vi "Make String Mermaid Safe.vi"(11 "Source CSM":string) -> (3 "result string":string)   [LabVIEW 2020, in "CSM Mermaid Support.lvlib"]
uses:
  CSM Mermaid Support.lvlib
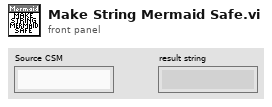
[diagram p1: front panel]
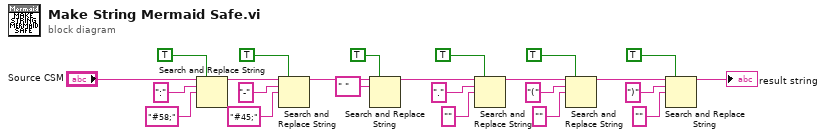
[diagram p0: block diagram]
diagram:
  n1 = Search and Replace String(replace all?=TRUE ("replace all? (F)"), input string="Source CSM", search string=":", replace string="#58;" ("search string")) -> (result string=w17:string)  [unwired: 4 in, 3 out]
  n2 = Search and Replace String(replace all?=TRUE ("replace all? (F)"), input string=w17, search string="-", replace string="#45;" ("search string")) -> (result string=w2:string)  [unwired: 4 in, 3 out]
  n3 = Search and Replace String(replace all?=TRUE ("replace all? (F)"), input string=w2, search string=" ") -> (result string=w1:string)  [unwired: 5 in, 3 out]
  n4 = Search and Replace String(replace all?=TRUE ("replace all? (F)"), input string=w1, search string=".", replace string="" ("search string")) -> (result string=w16:string)  [unwired: 4 in, 3 out]
  n5 = Search and Replace String(replace all?=TRUE ("replace all? (F)"), input string=w16, search string="(", replace string="" ("search string")) -> (result string=w6:string)  [unwired: 4 in, 3 out]
  n6 = Search and Replace String(replace all?=TRUE ("replace all? (F)"), input string=w6, search string=")", replace string="" ("search string")) -> (result string=→"result string":string)  [unwired: 4 in, 3 out]
